vi "VM Error Code Converter.vi"(2 "VM VI error code in":i32, 3 "VM Engine error code in":T1 items=["No error", "Invalid variable type", "Variable not found", "Variable already exists", "Invalid context handle", "Input error", "Invalid data format", "No history attached", "History already attached", "Invalid history parameters", "Wrong variable name", "Wrong alias name", "Non-unique alias", "Alias not found", "No alias associated", "Alias already associated", "Wrong context name", "Non-unique context name", "Context name not found", "Invalid parameter", "Generic error", "Memory Full", "Unrecognized LV error", "Unknown error code"]) -> (0 "VM Engine error code out":T1 items=["No error", "Invalid variable type", "Variable not found", "Variable already exists", "Invalid context handle", "Input error", "Invalid data format", "No history attached", "History already attached", "Invalid history parameters", "Wrong variable name", "Wrong alias name", "Non-unique alias", "Alias not found", "No alias associated", "Alias already associated", "Wrong context name", "Non-unique context name", "Context name not found", "Invalid parameter", "Generic error", "Memory Full", "Unrecognized LV error", "Unknown error code"], 1 "VM VI error code out":i32)   [LabVIEW 2021]
doc: "::: CalcExpress Toolkit :::\nCopyright (c) 2000-2026 Konstantin Shifershteyn. All rights reserved."
uses:
  cetypes.llb/VarMan Error Code.ctl
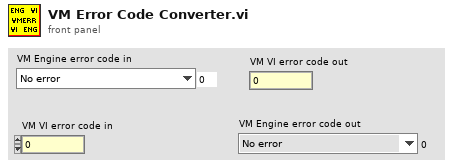
[diagram p1: front panel]
types:
  T1 = typedef "VarMan Error Code.ctl" = u16
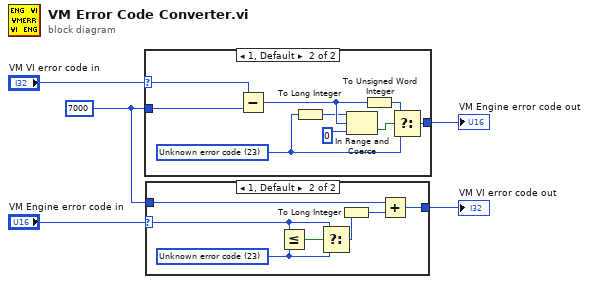
[diagram p0: block diagram]
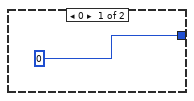
[diagram p2: hidden frame]
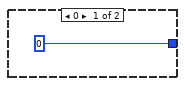
[diagram p3: hidden frame]
diagram:
  w2 = 7000
  n1 = case shown="1, Default" "VM VI error code in" {
    selector: "VM VI error code in" -> [_ w12]
    tunnel: [u16 0 ("VarMan Engine error") w14] -> w4
    tunnel: w2 -> [_ w7]
    frame 0 {
    }
    frame 1, Default {
      w8 = T1 23 items=["No error", "Invalid variable type", "Variable not found", "Variable already exists", "Invalid context handle", "Input error", "Invalid data format", "No history attached", "History already attached", "Invalid history parameters", "Wrong variable name", "Wrong alias name", "Non-unique alias", "Alias not found", "No alias associated", "Alias already associated", "Wrong context name", "Non-unique context name", "Context name not found", "Invalid parameter", "Generic error", "Memory Full", "Unrecognized LV error", "Unknown error code"] ("VarMan Engine error")
      n2 = Subtract(x=w12, y=w7) -> (x-y=w11:i32)
      n3 = To Long Integer(number=w8) -> (32bit integer=w9:i32)
      n4 = In Range and Coerce(upper limit=w9, x=w11, lower limit=0 ("lo")) -> (In Range?=w15:bool)  [unwired: 1 out]
      n5 = To Unsigned Word Integer(number=w11) -> (unsigned 16bit integer=w13:u16)
      n6 = Select(t=w13, s=w15, f=w8) -> (s? t:f=w14:T1)
    }
  }
  "VM Engine error code out" <- w4
  n7 = case shown="1, Default" "VM Engine error code in" {
    selector: "VM Engine error code in" -> [_ w18]
    tunnel: w2 -> [_ w23]
    tunnel: [0 w21] -> w1
    frame 0 {
    }
    frame 1, Default {
      w19 = T1 23 items=["No error", "Invalid variable type", "Variable not found", "Variable already exists", "Invalid context handle", "Input error", "Invalid data format", "No history attached", "History already attached", "Invalid history parameters", "Wrong variable name", "Wrong alias name", "Non-unique alias", "Alias not found", "No alias associated", "Alias already associated", "Wrong context name", "Non-unique context name", "Context name not found", "Invalid parameter", "Generic error", "Memory Full", "Unrecognized LV error", "Unknown error code"] ("VarMan Engine error")
      n8 = Less Or Equal?(x=w18, y=w19) -> (x <= y?=w20:bool)
      n9 = Select(t=w18, s=w20, f=w19) -> (s? t:f=w17:T1)
      n10 = To Long Integer(number=w17) -> (32bit integer=w22:i32)
      n11 = Add(x=w23, y=w22) -> (x+y=w21:i32)
    }
  }
  "VM VI error code out" <- w1
